vi "Get Sensor Size.vi"(8 "error in (no error)":errorcluster, 11 "Camera in":refnum<class "Camera.lvclass">) -> (0 "error out":errorcluster, 2 "Sensor Size":T1, 3 "Camera":refnum<class "Camera.lvclass">)   [LabVIEW 2020, in "Camera.lvclass"]
uses:
  Camera.lvclass
  Buffer/Image Size.ctl
  Camera.lvclass/Camera.ctl
  Buffer/Buffer.lvclass
  bin/gindustrialcam_32-1.dll
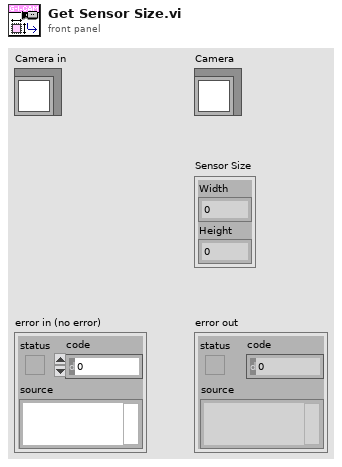
[diagram p1: front panel]
types:
  T1 = typedef "Buffer.lvclass/Image Size.ctl" = cluster{"Width":u16, "Height":u16}
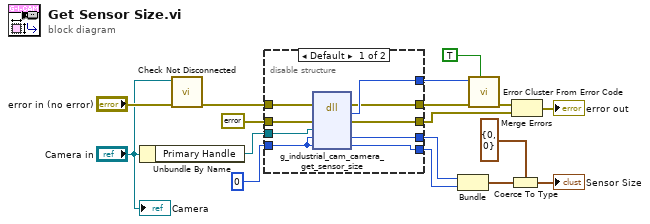
[diagram p0: block diagram]
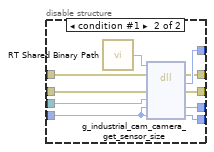
[diagram p2: hidden frame]
diagram:
  n1 = Unbundle By Name("Camera in") -> ("Primary Handle"=w12:refnum<data-value>)
  n2 = call "Check Not Disconnected.vi"("error in (no error)"="error in (no error)", "Camera in"="Camera in") -> ("error out"=w11:errorcluster)  [unwired: 9 in]
  n3 = disable-structure shown="Default" {
    disable-tunnel: errorcluster {"status"=FALSE, "code"=0, "source"=""} ("error constant") -> [w26 w36]
    disable-tunnel: w12 -> [w25 w35]
    disable-tunnel: w11 -> [w24 w34]
    disable-tunnel: [w23 w33] -> w9
    disable-tunnel: [w22 w32] -> w7
    disable-tunnel: [w21 w31] -> w6
    disable-tunnel: [w20 w30] -> w5
    disable-tunnel: [w19 w29] -> w4
    disable-tunnel: 0 ("width") -> [w18 w28]
    frame condition #0 (active) {
      n4 = dll-call lib="C:/serenial/lib/g-industrial-camera/LabVIEW/g_industrial_cam/bin/gindustrialcam_*-1.*" fn="g_industrial_cam_camera_get_sensor_size"(error in=w24, "err"=w26, "edvr"=w25, "width"=w18, "height"=w18) -> (error out=w21:errorcluster, "Mg_Error"=w22:i32, "err"=w23:errorcluster, "width"=w20:i32, "height"=w19:i32)  [unwired: 3 in, 1 out]
    }
    frame condition #1 {
      n5 = call "RT Shared Binary Path.vi"() -> ("Path"=w27:path)
      n6 = dll-call lib="C:/serenial/lib/g-industrial-camera/LabVIEW/g_industrial_cam/bin/gindustrialcam_*-1.*" fn="g_industrial_cam_camera_get_sensor_size"(path in=w27, error in=w34, "err"=w36, "edvr"=w35, "width"=w28, "height"=w28) -> (error out=w31:errorcluster, "Mg_Error"=w32:i32, "err"=w33:errorcluster, "width"=w30:i32, "height"=w29:i32)  [unwired: 2 in, 1 out]
    }
  }
  n7 = Bundle("width"=w5, "height"=w4) -> (w14:cluster{"width":i32, "height":i32})  [unwired: 1 in]
  n8 = call <vilib>:"Error Cluster From Error Code.vi"("show call chain? (False)"=TRUE, "error in (no error)"=w6, "error code (0)"=w7) -> ("error out"=w8:errorcluster)  [unwired: 6 in]
  n9 = Coerce To Type(0:w14, 1:T1 {"Width"=0, "Height"=0} ("Image Size")) -> (2:→"Sensor Size":T1)
  n10 = Merge Errors(w8, w9) -> (→"error out":errorcluster)
  "Camera" <- "Camera in"
